vi "VIH XML - File Array to-from XML String.vi"(6 "cmd (check)":enum16{"check", "parse", "format"}(ring), 8 "error in":errorcluster, 10 "Files in":path[](array[path]), 11 "XML in":string) -> (0 "error out":errorcluster, 1 "available":bool, 2 "Files out":path[](array[path]), 3 "XML out":string)   [LabVIEW 2014]
doc: "::: VI Helpeks :::\nCopyright (c) 2000-2026 Konstantin Shifershteyn. All rights reserved."
uses:
  <vilib>/xml/Close Reference(Node).vi
  <vilib>/xml/NI_XML.lvlib
  <resource>/objmgr/DOMUserDefRef.rc
panel:
  # "VI Helpeks\nCopyright (c) 2012-2026 Konstantin Shifershteyn"
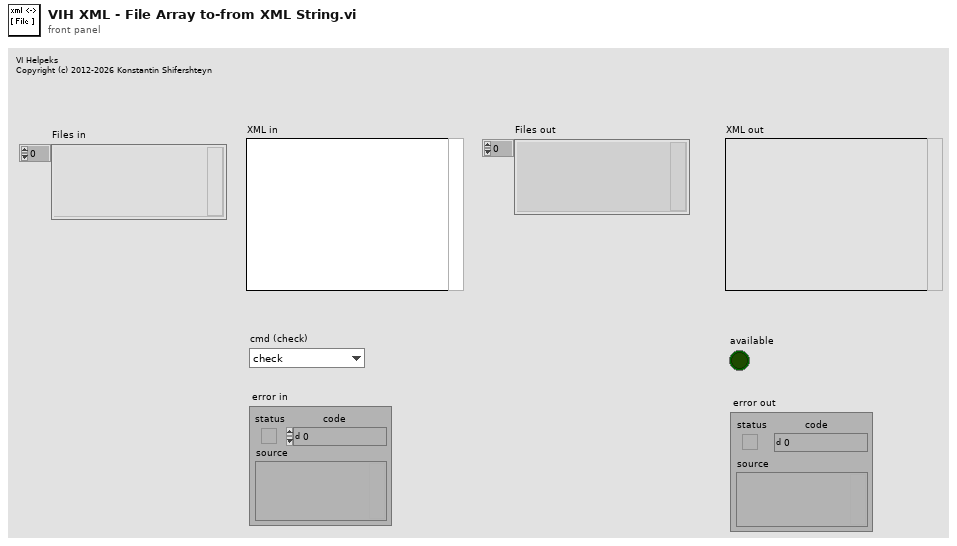
[diagram p1: front panel]
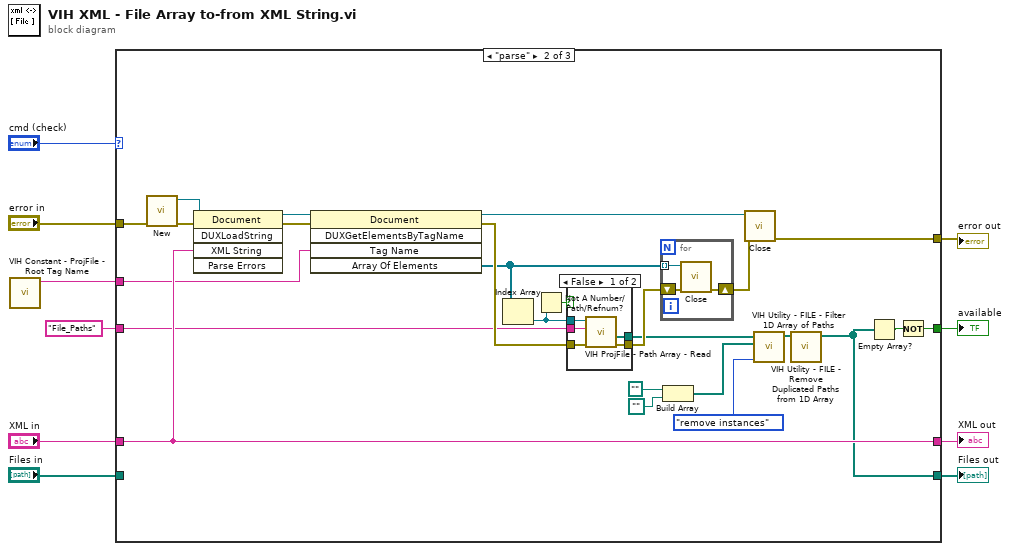
[diagram p0: block diagram]
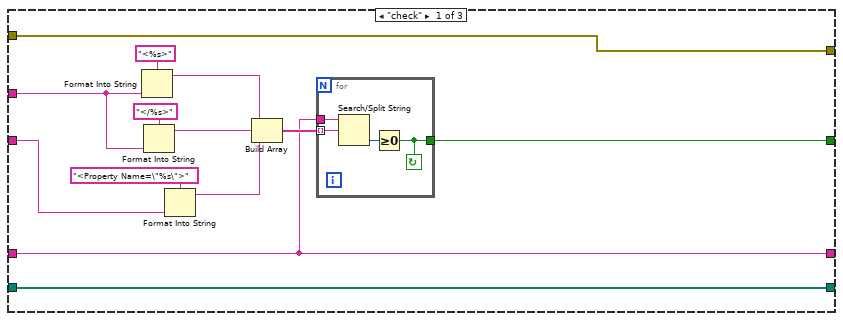
[diagram p2: hidden frame]
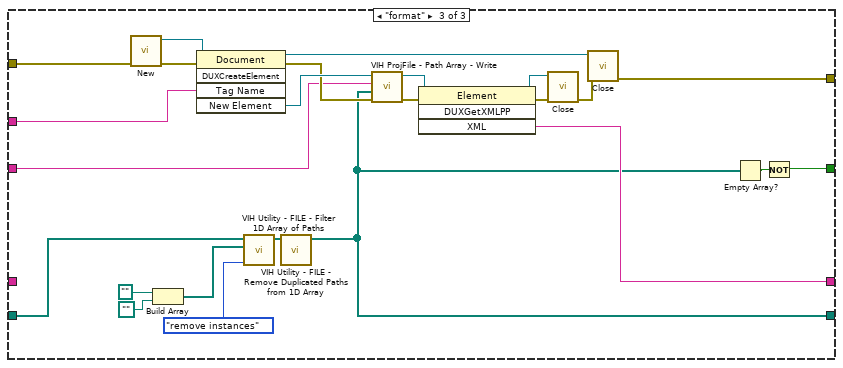
[diagram p4: hidden frame]
diagram:
  n1 = call "VIH Constant - ProjFile - Root Tag Name.vi"() -> ("Tag Name"=w1:string)  [unwired: 11 in]
  n2 = case shown="\"parse\"" "cmd (check)" {
    tunnel: "error in" -> [w23 w41 w75]
    tunnel: "Files in" -> [w22 _ w65]
    tunnel: [w23 w40 w74] -> w7
    tunnel: [w17 w39 w73] -> w6
    tunnel: [w22 w28 w62] -> w5
    tunnel: "XML in" -> [w17 w39 _]
    tunnel: w1 -> [w13 w38 w72]
    tunnel: "File_Paths" ("Property Name") -> [w11 w37 w71]
    tunnel: [w18 w36 w63] -> w2
    frame "check" {
      n3 = Format Into String(format string="<%s>", w13) -> (resulting string=w16:string)  [unwired: 2 in, 1 out]
      n4 = Format Into String(format string="</%s>", w13) -> (resulting string=w15:string)  [unwired: 2 in, 1 out]
      n5 = Format Into String(format string="<Property Name=\"%s\">", w11) -> (resulting string=w12:string)  [unwired: 2 in, 1 out]
      n6 = Build Array(w16, w15, w12) -> (w21:string[])
      n7 = for {
        tunnel: w21 -> [w25] mode=indexing
        tunnel: [w26] -> w18
        tunnel: w17 -> [w24]
        stop <- w26 continue-if-true
        n8 = Search/Split String(string=w24, search string/char (-)=w25) -> (offset of match=w27:i32)  [unwired: 1 in, 2 out]
        n9 = Greater Or Equal To 0?(x=w27) -> (x >= 0?=w26:bool)
      }
    }
    frame "parse" {
      n10 = call <vilib>:"New.vi"("error in (no error)"=w41) -> ("error out"=w51:errorcluster, "DOM document out"=w52:refnum<k20>)  [unwired: 7 in]
      n11 = invoke class="Document" method="DUXLoadString"(reference=w52, error in=w51, "XML String"=w39) -> (reference out=w49:refnum<k20>, error out=w48:errorcluster)  [unwired: 2 in, 3 out]
      n12 = invoke class="Document" method="DUXGetElementsByTagName"(reference=w49, error in=w48, "Tag Name"=w38) -> (reference out=w46:refnum<k20>, error out=w47:errorcluster, "Array Of Elements"=w45:refnum<k20>[])  [unwired: 2 in, 2 out]
      n13 = Index Array(array=w45) -> (element=w43:refnum<k20>)  [unwired: 1 in]
      n14 = Not A Number/Path/Refnum?(number/path/refnum=w43) -> (NaN/Path/Refnum?=w42:bool)
      n15 = case shown="False" w42 {
        tunnel: w37 -> [w54 _]
        tunnel: w47 -> [w57 w58]
        tunnel: [w56 w58] -> w44
        tunnel: w43 -> [w55 _]
        tunnel: [w53 _] -> w29
        frame False {
          n16 = call "VIH ProjFile - Path Array - Read.vi"("error in"=w57, "Property Name"=w54, "XML Parent Item"=w55) -> ("error out"=w56:errorcluster, "Files"=w53:path[])  [unwired: 6 in, 1 out]
        }
        frame True {
        }
      }
      n17 = for {
        tunnel: w45 -> [w60] mode=indexing
        shift-right: [w61] -> w50
        shift-left: w44 -> [w59]
        n18 = call-poly <vilib>:"Close.vi"("error in (no error)"=w59, "node"=w60) -> ("error out"=w61:errorcluster)  [unwired: 7 in]
      }
      n19 = Build Array(path "", path "") -> (w34:path[])
      n20 = call-poly <vilib>:"Close.vi"("error in (no error)"=w50, "node"=w46) -> ("error out"=w40:errorcluster)  [unwired: 7 in]
      n21 = call "VIH Utility - FILE - Filter 1D Array of Paths.vi"("Action (keep instances)"=enum16{"keep instances", "remove instances"}."remove instances", "Instances"=w34, "Paths in"=w29) -> ("Paths out"=w30:path[])  [unwired: 4 in]
      n22 = call "VIH Utility - FILE - Remove Duplicated Paths from 1D Array.vi"("Array in"=w30) -> ("Array out"=w28:path[])  [unwired: 9 in, 1 out]
      n23 = Empty Array?(array=w28) -> (empty?=w35:bool)
      n24 = Not(x=w35) -> (.not. x?=w36:bool)
    }
    frame "format" {
      n25 = call <vilib>:"New.vi"("error in (no error)"=w75) -> ("error out"=w81:errorcluster, "DOM document out"=w84:refnum<k20>)  [unwired: 7 in]
      n26 = Build Array(path "", path "") -> (w70:path[])
      n27 = invoke class="Document" method="DUXCreateElement"(reference=w84, error in=w81, "Tag Name"=w72) -> (reference out=w82:refnum<k20>, error out=w83:errorcluster, "New Element"=w85:refnum<k20>)  [unwired: 2 in, 2 out]
      n28 = call "VIH Utility - FILE - Filter 1D Array of Paths.vi"("Action (keep instances)"=enum16{"keep instances", "remove instances"}."remove instances", "Instances"=w70, "Paths in"=w65) -> ("Paths out"=w66:path[])  [unwired: 4 in]
      n29 = call "VIH Utility - FILE - Remove Duplicated Paths from 1D Array.vi"("Array in"=w66) -> ("Array out"=w62:path[])  [unwired: 9 in, 1 out]
      n30 = call "VIH ProjFile - Path Array - Write.vi"("error in"=w83, "Paths"=w62, "Property Name"=w71, "XML Parent Item"=w85) -> ("error out"=w77:errorcluster, "dup XML Parent Item"=w76:refnum<k20>)  [unwired: 6 in]
      n31 = invoke class="Element" method="DUXGetXMLPP"(reference=w76, error in=w77) -> (reference out=w79:refnum<k20>, error out=w78:errorcluster, "XML"=w73:string)  [unwired: 2 in, 1 out]
      n32 = call-poly <vilib>:"Close.vi"("error in (no error)"=w78, "node"=w79) -> ("error out"=w80:errorcluster)  [unwired: 7 in]
      n33 = call-poly <vilib>:"Close.vi"("error in (no error)"=w80, "node"=w82) -> ("error out"=w74:errorcluster)  [unwired: 7 in]
      n34 = Empty Array?(array=w62) -> (empty?=w64:bool)
      n35 = Not(x=w64) -> (.not. x?=w63:bool)
    }
  }
  "Files out" <- w5
  "XML out" <- w6
  "error out" <- w7
  "available" <- w2
